vi "lab2_3_subvi1.vi"(8 "Acc in":i16, 11 "Acc prev":i16) -> (0 "Acceleration Max":i16, 3 "Acceleration Now":i16)   [LabVIEW 2026]
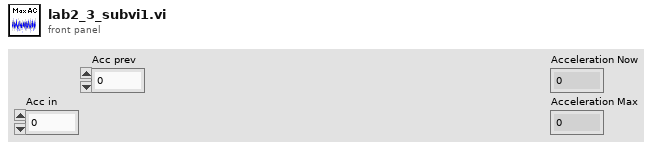
[diagram p1: front panel]
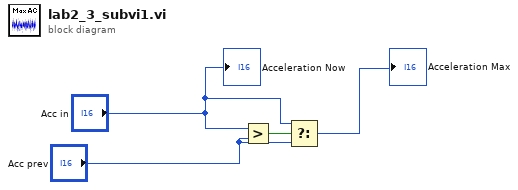
[diagram p0: block diagram]
diagram:
  n1 = Greater?(x="Acc in", y="Acc prev") -> (0:w4:bool)
  n2 = Select(t="Acc in", s=w4, f="Acc prev") -> (s? t:f=→"Acceleration Max":i16)
  "Acceleration Now" <- "Acc in"
